vi "Init.vi"(8 "error in (no error)":errorcluster, 10 "Image Refnum":refnum<vi>, 11 "ImageHandler:DT-ImageHandler in":refnum<class "DT-ImageHandler.lvclass">) -> (0 "error out":errorcluster, 3 "ImageHandler:DT-ImageHandler out":refnum<class "DT-ImageHandler.lvclass">)   [LabVIEW 2022 SP3, in "ImageHandler.lvlib" / "DT-ImageHandler.lvclass"]
uses:
  DT-ImageHandler.lvclass
  DT-ImageHandler.lvclass/DT-ImageHandler.ctl
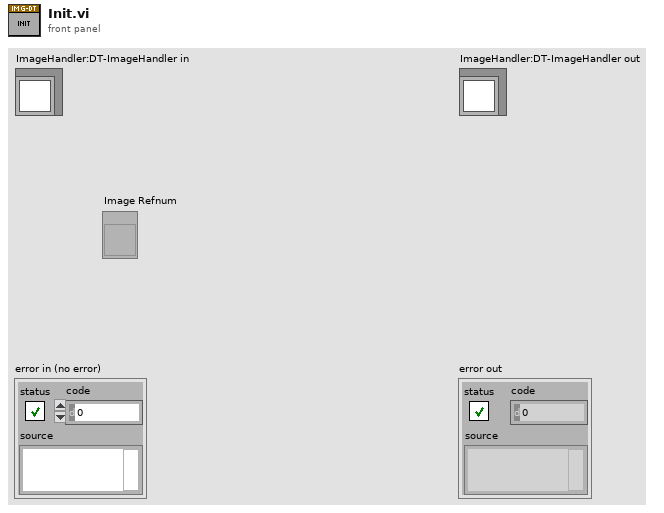
[diagram p1: front panel]
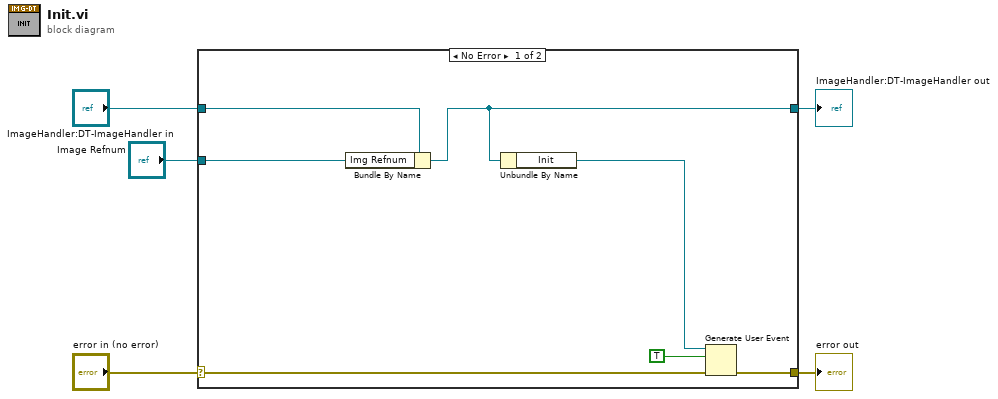
[diagram p0: block diagram]
diagram:
  n1 = case shown="No Error" "error in (no error)" {
    selector: "error in (no error)" -> [w12 w14]
    tunnel: [w10 w14] -> w4
    tunnel: [w7 w13] -> w2
    tunnel: "ImageHandler:DT-ImageHandler in" -> [w11 w13]
    tunnel: "Image Refnum" -> [w6 _]
    frame No Error {
      n2 = Bundle By Name(cluster=w11, "Img Refnum"=w6) -> (w7:refnum<class "DT-ImageHandler.lvclass">)
      n3 = Unbundle By Name(w7) -> ("Init"=w9:refnum<user-event>)
      n4 = Generate User Event(user event=w9, event data cluster=TRUE ("event data"), error in=w12) -> (error out=w10:errorcluster)  [unwired: 1 in, 1 out]
    }
    frame Error {
    }
  }
  "error out" <- w4
  "ImageHandler:DT-ImageHandler out" <- w2
